vi "Mandelbrot_LabVIEW.vi"(7 "Max_iter":i32=4000, 8 "Zoom":dbl=5e-11, 9 "y":dbl=0.13182590420533, 10 "x":dbl=-0.743643887037151, 11 "Resolution":i32=1000) -> (0 "Exec Time":dbl=3.6367448000000877, 3 "Mandelbrot Graph":i16[][](graph))   [LabVIEW 2020]
uses:
  250ad98c-c819-4240-bb72-613057cdb05b.vi
  8fc4144a-0758-458b-88ac-401a6681cd74.vi
  <vilib>/Analysis/1siggen.llb/Ramp Pattern by Samples.vi
  <vilib>/Utility/High Resolution Relative Seconds.vi
  <vilib>/Analysis/NI_AALBase.lvlib
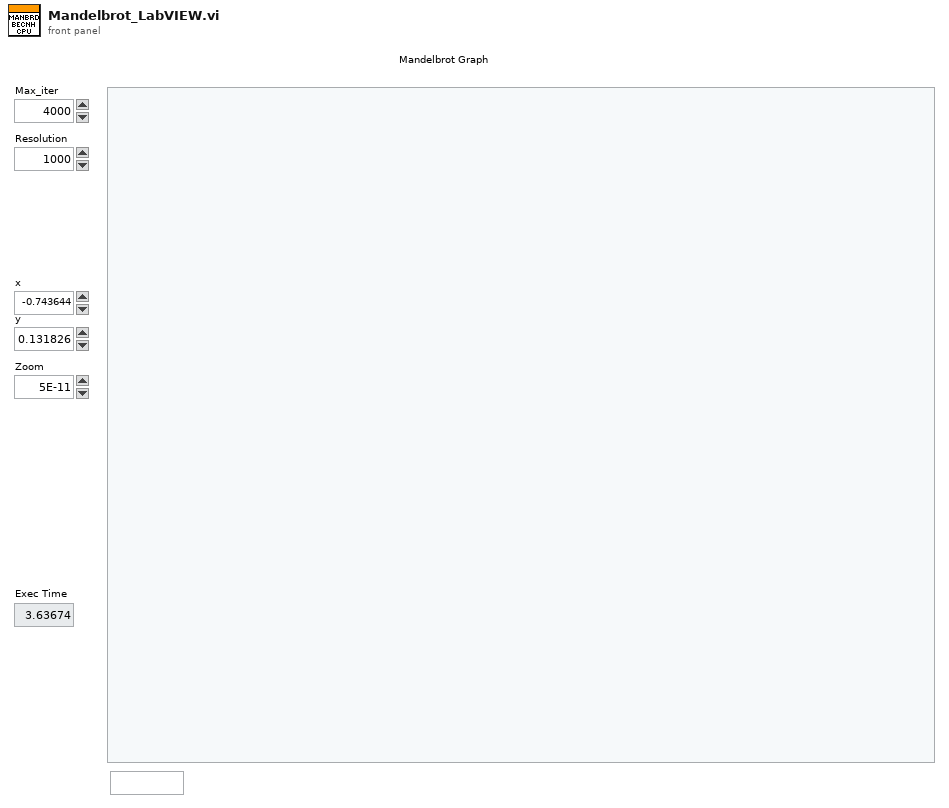
[diagram p1: front panel]
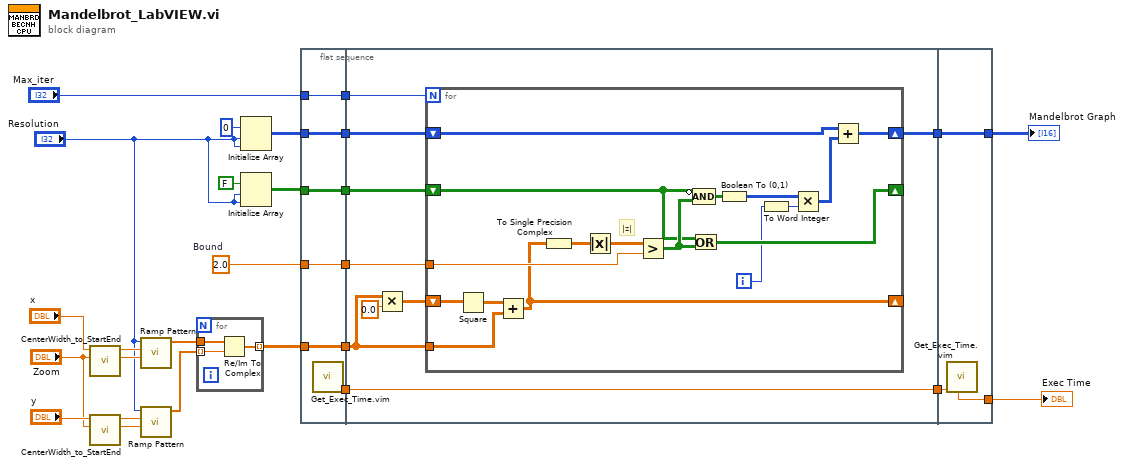
[diagram p0: block diagram]
diagram:
  w12 = sgl 2.0  # Bound
  n1 = call "CenterWidth_to_StartEnd.vi"("width"="Zoom", "Center"="x") -> ("Start"=w18:dbl, "End"=w19:dbl)  [unwired: 8 in]
  n2 = call "CenterWidth_to_StartEnd.vi"("width"="Zoom", "Center"="y") -> ("Start"=w14:dbl, "End"=w15:dbl)  [unwired: 8 in]
  n3 = call-poly <vilib>:"Ramp Pattern.vi"("start"=w18, "end"=w19, "samples"="Resolution") -> ("Ramp Pattern"=w17:dbl[])  [unwired: 7 in, 1 out]
  n4 = call-poly <vilib>:"Ramp Pattern.vi"("start"=w14, "end"=w15, "samples"="Resolution") -> ("Ramp Pattern"=w16:dbl[])  [unwired: 7 in, 1 out]
  n5 = for {
    tunnel: w16 -> [w29] mode=indexing
    tunnel: w17 -> [w30]
    tunnel: [w28] -> w13 mode=indexing
    n6 = Re/Im To Complex(1:w29, 2:w30) -> (0:w28:cdb[])
  }
  n7 = Initialize Array(i16 0 ("element"), "Resolution", "Resolution") -> (w10:i16[][])
  n8 = Initialize Array(FALSE, "Resolution", "Resolution") -> (w8:bool[][])
  n9 = flat-sequence {
    tunnel: w13 -> [w34]
    tunnel: w8 -> [w35]
    tunnel: "Max_iter" -> [w36]
    tunnel: [w36] -> w27
    tunnel: [w35] -> w26
    tunnel: [w34] -> w25
    tunnel: [w33] -> w24
    tunnel: [w32] -> w23
    tunnel: w10 -> [w32]
    tunnel: [w31] -> w22
    tunnel: w12 -> [w31]
    tunnel: w27 -> [w45]
    tunnel: w26 -> [w37]
    tunnel: w25 -> [w44]
    tunnel: [w41] -> w21
    tunnel: w24 -> [w41]
    tunnel: w23 -> [w38]
    tunnel: [w39] -> w20
    tunnel: w22 -> [w40]
    tunnel: w21 -> [w65]
    tunnel: [w64] -> w7
    tunnel: [w63] -> w1
    tunnel: w20 -> [w63]
    frame #0 {
      n10 = call "Get_Exec_Time.vim"() -> ("T(n)"=w33:dbl)  [unwired: 7 in, 2 out]
    }
    frame #1 {
      n11 = Multiply(x=w44, y=sgl 0.0 ("start")) -> (x*y=w43:cdb[][])
      n12 = for {
        N: w45 -> [_]
        shift-right: [w51] -> _
        shift-left: w43 -> [w52]
        tunnel: w44 -> [w59]
        shift-right: [w62] -> w39
        shift-left: w38 -> [w55]
        tunnel: w40 -> [w60]
        shift-right: [w61] -> _
        shift-left: w37 -> [w47]
        i -> [w53]
        # "|z|"
        n13 = Square(x=w52) -> (x^2=w48:cdb[][])
        n14 = Add(x=w48, y=w59) -> (x+y=w51:cdb[][])
        n15 = To Single Precision Complex(1:w51) -> (0:w49:csg[][])
        n16 = Absolute Value(x=w49) -> (abs(x)=w50:sgl[][])
        n17 = Greater?(x=w50, y=w60) -> (0:w58:bool[][])
        n18 = Or(x=w47, y=w58) -> (x .or. y?=w61:bool[][])
        n19 = Compound Arithmetic op=AND(invert w47, w58) -> (w57:bool[][])
        n20 = Boolean To (0,1)(Boolean=w57) -> (0, 1=w54:i16[][])
        n21 = To Word Integer(number=w53) -> (16bit integer=w46:i16)
        n22 = Multiply(x=w54, y=w46) -> (x*y=w56:i16[][])
        n23 = Add(x=w55, y=w56) -> (x+y=w62:i16[][])
      }
    }
    frame #2 {
      n24 = call "Get_Exec_Time.vim"("T(n-1)"=w65) -> ("dT"=w64:dbl)  [unwired: 6 in, 2 out]
    }
  }
  "Mandelbrot Graph" <- w1
  "Exec Time" <- w7
